vi "update channel names to match tags.vi"(8 "error in":errorcluster, 10 "TEC in":refnum<class "TEC configuration.lvclass">, 11 "engine configuration in":refnum<class "engine configuration.lvclass">) -> (0 "error out":errorcluster, 2 "TEC out":refnum<class "TEC configuration.lvclass">, 3 "engine configuration out":refnum<class "engine configuration.lvclass">)   [LabVIEW 2013, in "TEC editor node.lvclass"]
uses:
  TEC editor node.lvclass
  configuration/TEC configuration.lvclass
  <vilib>/NI/Module Execution Interface/Engine Configuration/engine configuration.lvclass
  <vilib>/NI/Configuration Framework/serializable configuration/NISE_CEF_serializable configuration.lvclass/NISE_CEF_serializable configuration.ctl
  configuration/TEC configuration.lvclass/TEC configuration.ctl
  <vilib>/NI/Tag Bus/tag/tag descriptor.lvclass/tag descriptor.ctl
  <vilib>/NI/Tag Bus/tag/write tag name.vi
  <vilib>/NI/Tag Bus/tag/read tag name.vi
  <vilib>/NI/Configuration Framework/serializable configuration/Read UID.vi
  configuration/Read channels.vi
  <vilib>/Utility/LVClass/Get LV Class Name.vi
  <vilib>/NI/Configuration Framework/error generator/NISE_error generator.vi
  <vilib>/NI/Tag Bus Module Framework/channel/TBM channel.lvclass
  <vilib>/NI/Tag Bus/tag/tag descriptor.lvclass
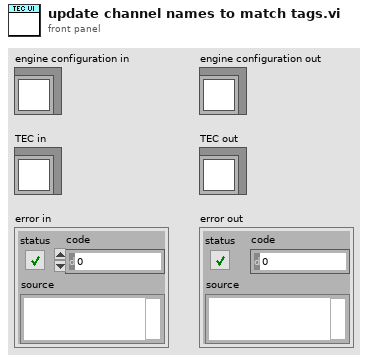
[diagram p1: front panel]
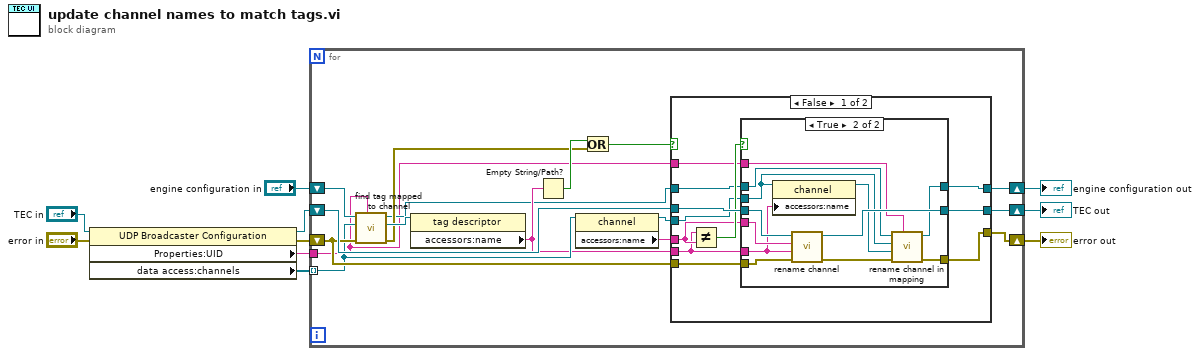
[diagram p0: block diagram]
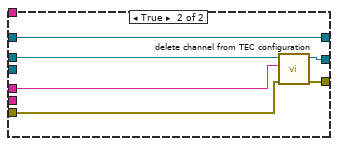
[diagram p3: hidden frame]
diagram:
  n1 = property class="UDP Broadcaster Configuration"(reference="TEC in", error in="error in") -> (reference out=w3:refnum<class "TEC configuration.lvclass">, error out=w2:errorcluster, "Properties:UID"=w6:string, "data access:channels"=w1:refnum<class "TBM channel.lvclass">[])
  n2 = for {
    tunnel: w1 -> [w18] mode=indexing
    shift-right: [w13] -> w7
    shift-left: "engine configuration in" -> [w26]
    shift-right: [w23] -> w4
    shift-left: w3 -> [w21]
    tunnel: w6 -> [w12]
    shift-right: [w22] -> w5
    shift-left: w2 -> [w19]
    n3 = call <vilib>:"find tag mapped to channel.vi"("owner"=w12, "error in"=w19, "channel"=w18, "engine configuration in"=w26) -> ("error out"=w17:errorcluster, "tag"=w25:refnum<class "tag descriptor.lvclass">, "engine configuration out"=w14:refnum<class "engine configuration.lvclass">)  [unwired: 5 in]
    n4 = property class="tag descriptor"(reference=w25) -> ("accessors:name"=w15:string)  [unwired: 1 in, 2 out]
    n5 = Empty String/Path?(string/path=w15) -> (empty?=w24:bool)
    n6 = property class="channel"(reference=w18) -> (reference out=w11:refnum<class "TBM channel.lvclass">, "accessors:name"=w16:string)  [unwired: 1 in, 1 out]
    n7 = Or(x=w24, y=w17) -> (x .or. y?=w20:bool)
    n8 = case shown="False" w20 {
      tunnel: [w34 w58] -> w23
      tunnel: [w37 w57] -> w22
      tunnel: w19 -> [w36 w56]
      tunnel: w21 -> [w35 w55]
      tunnel: w16 -> [w32 w54]
      tunnel: w15 -> [w31 _]
      tunnel: w14 -> [w30 w53]
      tunnel: [w29 w53] -> w13
      tunnel: w12 -> [w28 _]
      tunnel: w11 -> [w27 _]
      frame False {
        n9 = Not Equal?(x=w31, y=w32) -> (x != y?=w33:bool)
        n10 = case shown="True" w33 {
          tunnel: [w40 w45] -> w37
          tunnel: w36 -> [w40 w52]
          tunnel: w35 -> [w39 w51]
          tunnel: [w39 w50] -> w34
          tunnel: w32 -> [_ w49]
          tunnel: w31 -> [_ w41]
          tunnel: w30 -> [w38 w48]
          tunnel: [w38 w47] -> w29
          tunnel: w28 -> [_ w44]
          tunnel: w27 -> [_ w43]
          frame False {
          }
          frame True {
            n11 = property class="channel"(reference=w43, "accessors:name"=w41) -> (reference out=w42:refnum<class "TBM channel.lvclass">)  [unwired: 1 in, 1 out]
            n12 = call "rename channel.vi"("error in"=w52, "new name"=w41, "old name"=w49, "TEC configuration in"=w51) -> ("error out"=w46:errorcluster, "TEC configuration out"=w50:refnum<class "TEC configuration.lvclass">)  [unwired: 6 in]
            n13 = call <vilib>:"rename channel in mapping.vi"("owner ID"=w44, "error in"=w46, "new channel"=w42, "old channel"=w43, "engine configuration in"=w48) -> ("error out"=w45:errorcluster, "engine configuration out"=w47:refnum<class "engine configuration.lvclass">)  [unwired: 5 in]
          }
        }
      }
      frame True {
        n14 = call "delete channel from TEC configuration.vi"("error in"=w56, "channel to delete"=w54, "TEC configuration in"=w55) -> ("error out"=w57:errorcluster, "TEC configuration out"=w58:refnum<class "TEC configuration.lvclass">)  [unwired: 7 in]
      }
    }
  }
  "engine configuration out" <- w7
  "error out" <- w5
  "TEC out" <- w4
